vi "getSerializedData.vi"(0 "reference":refnum<class "PackageNode.lvclass">, 5 "error in (no error)":errorcluster) -> (14 "reference out":refnum<class "PackageNode.lvclass">, 15 "parent":refnum<class "AbstractNode.lvclass">, 16 "children":refnum<class "AbstractNode.lvclass">[](array[class]), 17 "xmlOut":string, 19 "error out":errorcluster)   [LabVIEW 2020, in "PackageNode.lvclass"]
doc: "getSerializedData"
uses:
  <resource>/Framework/Providers/Open_GDS/UML/PackageNode_class/PackageNode.lvclass
  C:/Program Files (x86)/National Instruments/LabVIEW 2020/resource/Framework/Providers/Open_GDS/UML/RectangularNode_class/RectangularNode.lvclass
  C:/Program Files (x86)/National Instruments/LabVIEW 2020/resource/Framework/Providers/Open_GDS/UML/AbstractNode_class/AbstractNode.lvclass
  <resource>/Framework/Providers/Open_GDS/UML/AbstractNode_class/AbstractNode.lvclass
  <resource>/Framework/Providers/Open_GDS/UML/General/Rectangle/Rectangle Rectangle2D.ctl
  <resource>/Framework/Providers/Open_GDS/UML/MultiLineString_class/MultiLineString.lvclass
  <resource>/Framework/Providers/Open_GDS/UML/RectangularNode_class/RectangularNode.lvclass
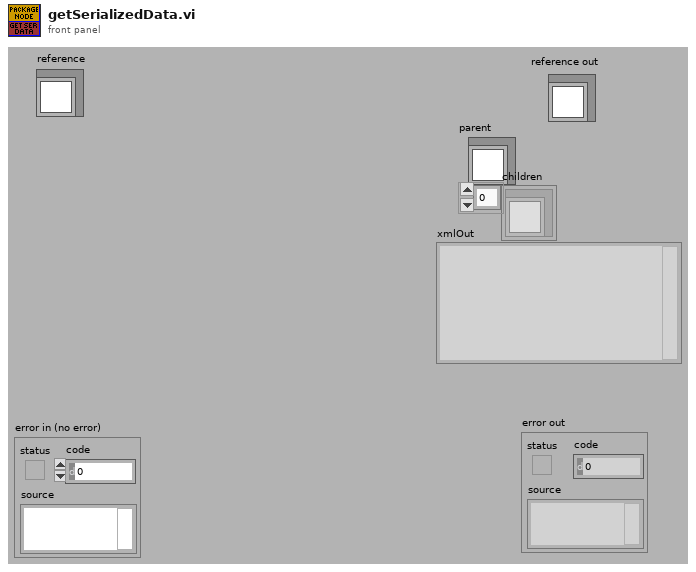
[diagram p1: front panel]
types:
  T1 = typedef "Rectangle Rectangle2D.ctl" = cluster{"x":dbl, "y":dbl, "width":dbl, "height":dbl}
  T2 = cluster{"Base class":cluster{"Base class":cluster{"parent":refnum<k1>, "children":refnum<k1>[], "Hidden":bool}, "bounds":T1}, "name":string, "contents":refnum<k1>, "DEFAULT_TOP_WIDTH":i32, "DEFAULT_TOP_HEIGHT":i32, "DEFAULT_WIDTH":i32, "DEFAULT_HEIGHT":i32, "NAME_GAP":i32, "XGAP":i32, "YGAP":i32, "Collapsed":bool, "Note color":u32, "Justification":u16}
  T3 = typedef "PackageNode.lvclass/ObjectAttributes.ctl" = cluster{"name":string, "contents":refnum<class "MultiLineString.lvclass">, "DEFAULT_TOP_WIDTH":i32, "DEFAULT_TOP_HEIGHT":i32, "DEFAULT_WIDTH":i32, "DEFAULT_HEIGHT":i32, "NAME_GAP":i32, "XGAP":i32, "YGAP":i32, "Collapsed":bool, "Note color":u32, "Justification":u16}
  T4 = typedef "RectangularNode.lvclass/ObjectAttributes.ctl" = cluster{"bounds":T1}
  T5 = typedef "AbstractNode.lvclass/ObjectAttributes.ctl" = cluster{"parent":refnum<class "AbstractNode.lvclass">, "children":refnum<class "AbstractNode.lvclass">[], "Hidden":bool}
  T6 = cluster{"Attributes":cluster{"Base class":cluster{"Base class":cluster{"parent":refnum<k1>, "children":refnum<k1>[], "Hidden":bool}, "bounds":T1}, "name":string, "contents":refnum<k1>, "DEFAULT_TOP_WIDTH":i32, "DEFAULT_TOP_HEIGHT":i32, "DEFAULT_WIDTH":i32, "DEFAULT_HEIGHT":i32, "NAME_GAP":i32, "XGAP":i32, "YGAP":i32, "Collapsed":bool, "Note color":u32, "Justification":u16}, "text":string}
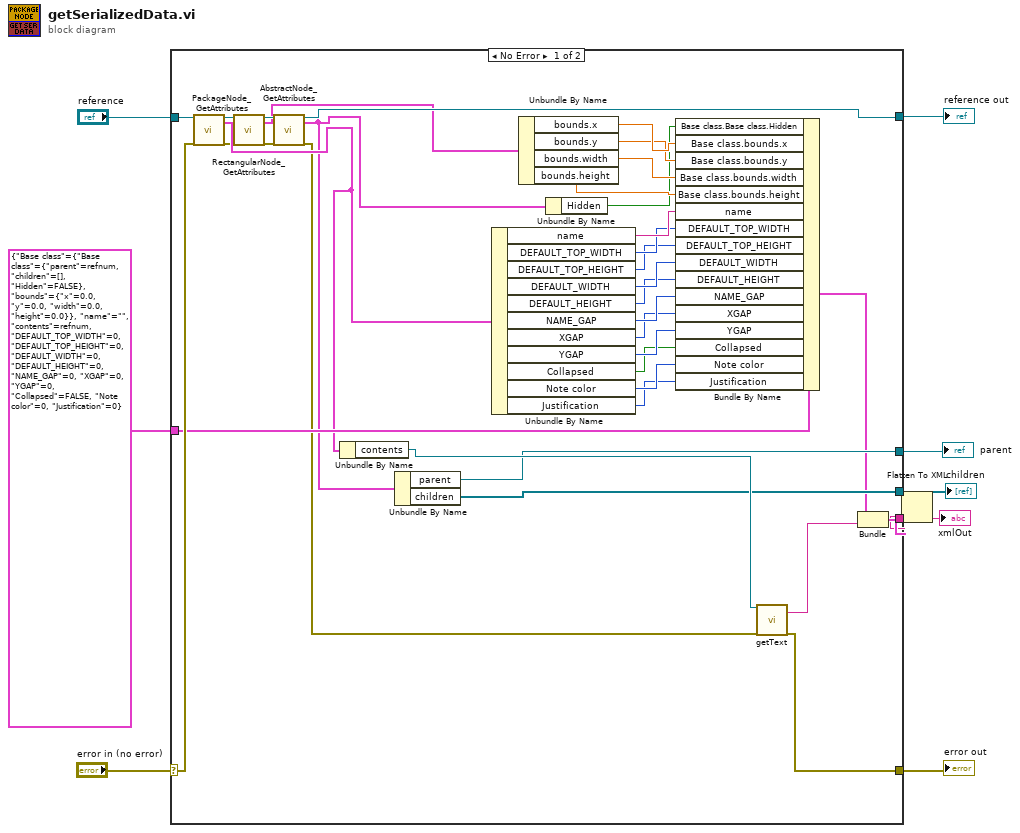
[diagram p0: block diagram]
diagram:
  n1 = case shown="No Error" "error in (no error)" {
    selector: "error in (no error)" -> [w44 w45]
    tunnel: "reference" -> [w43 w46]
    tunnel: [w39 w45] -> w6
    tunnel: [w11 w46] -> w5
    tunnel: [w38 _] -> w4
    tunnel: [w37 _] -> w3
    tunnel: [w36 _] -> w2
    tunnel: T2 {"Base class"={"Base class"={"parent"=refnum, "children"=[], "Hidden"=FALSE}, "bounds"={"x"=0.0, "y"=0.0, "width"=0.0, "height"=0.0}}, "name"="", "contents"=refnum, "DEFAULT_TOP_WIDTH"=0, "DEFAULT_TOP_HEIGHT"=0, "DEFAULT_WIDTH"=0, "DEFAULT_HEIGHT"=0, "NAME_GAP"=0, "XGAP"=0, "YGAP"=0, "Collapsed"=FALSE, "Note color"=0, "Justification"=0} ("Attributes") -> [w28 _]
    frame No Error {
      n2 = call <resource>:"PackageNode_GetAttributes.vi"("reference in"=w43, "error in (no error)"=w44) -> ("reference out"=w16:refnum<class "PackageNode.lvclass">, "Data"=w17:T3, "error out"=w15:errorcluster)  [unwired: 1 in, 14 out]
      n3 = call <resource>:"RectangularNode_GetAttributes.vi"("reference in"=w16, "error in (no error)"=w15) -> ("reference out"=w14:refnum<class "PackageNode.lvclass">, "Data"=w9:T4, "error out"=w13:errorcluster)  [unwired: 14 in, 1 out]
      n4 = call <resource>:"AbstractNode_GetAttributes.vi"("reference in"=w14, "error in (no error)"=w13) -> ("reference out"=w11:refnum<class "PackageNode.lvclass">, "Data"=w10:T5, "error out"=w12:errorcluster)  [unwired: 14 in, 1 out]
      n5 = Unbundle By Name(w17) -> ("contents"=w40:refnum<class "MultiLineString.lvclass">)
      n6 = Unbundle By Name(w10) -> ("parent"=w38:refnum<class "AbstractNode.lvclass">, "children"=w37:refnum<class "AbstractNode.lvclass">[])
      n7 = Unbundle By Name(w17) -> ("name"=w34:string, "DEFAULT_TOP_WIDTH"=w33:i32, "DEFAULT_TOP_HEIGHT"=w32:i32, "DEFAULT_WIDTH"=w31:i32, "DEFAULT_HEIGHT"=w30:i32, "NAME_GAP"=w24:i32, "XGAP"=w23:i32, "YGAP"=w22:i32, "Collapsed"=w21:bool, "Note color"=w19:u32, "Justification"=w18:u16)
      n8 = Unbundle By Name(w9) -> ("bounds.x"=w27:dbl, "bounds.y"=w26:dbl, "bounds.width"=w25:dbl, "bounds.height"=w35:dbl)
      n9 = Unbundle By Name(w10) -> ("Hidden"=w20:bool)
      n10 = Bundle By Name(cluster=w28, "Base class.Base class.Hidden"=w20, "Base class.bounds.x"=w27, "Base class.bounds.y"=w26, "Base class.bounds.width"=w25, "Base class.bounds.height"=w35, "name"=w34, "DEFAULT_TOP_WIDTH"=w33, "DEFAULT_TOP_HEIGHT"=w32, "DEFAULT_WIDTH"=w31, "DEFAULT_HEIGHT"=w30, "NAME_GAP"=w24, "XGAP"=w23, "YGAP"=w22, "Collapsed"=w21, "Note color"=w19, "Justification"=w18) -> (w29:T2)
      n11 = call-dynamic "getText.vi"("reference"=w40, "error in (no error)"=w12) -> ("text"=w41:string, "error out"=w39:errorcluster)  [unwired: 16 out]
      n12 = Bundle("Attributes"=w29, "text"=w41) -> (w42:T6)  [unwired: 1 out]
      n13 = Flatten To XML(6:w42) -> (2:w36:string)
    }
    frame Error {
    }
  }
  "reference out" <- w5
  "error out" <- w6
  "parent" <- w4
  "children" <- w3
  "xmlOut" <- w2
